vi "06a-arrays.vi"() -> ()   [LabVIEW 2018, in "LV2Julia_examples.lvlib"]
uses:
  LV2Julia_examples.lvlib
  LV2Julia_core/VIs/Server or client state.ctl
  LV2Julia_core/VIs/detailed error info.ctl
  LV2Julia_core/VIs/StackFrame.ctl
  LV2Julia_core/VIs/Commands.ctl
  72a46192-383e-4ee5-9465-71670922b82a.vi
  ef5408d4-6538-41d1-b296-fda05a71e4b0.vi
  5eac2bf2-d9fb-4bf1-948e-1ebc05516bc9.vi
  e4efb182-1b04-4d49-96a3-1defebd055ea.vi
  ebebf057-8b7e-42d1-8726-0ed76f361650.vi
  72a46192-383e-4ee5-9465-71670922b82a.vi/b0d408ed-daf5-454d-9ecc-f8af6744abda.vi
  ef5408d4-6538-41d1-b296-fda05a71e4b0.vi/f9ecc56d-b53d-412a-9af8-1c97b46c8685.vi
  5eac2bf2-d9fb-4bf1-948e-1ebc05516bc9.vi/a7715925-f8ed-4395-a6c4-c44ea2ed31c4.vi
  e4efb182-1b04-4d49-96a3-1defebd055ea.vi/824be71f-c5ad-4223-87c9-7cdbbdd09736.vi
  e4efb182-1b04-4d49-96a3-1defebd055ea.vi/40be3533-35a9-4e4c-8722-5f4375dd3b08.vi
  e4efb182-1b04-4d49-96a3-1defebd055ea.vi/65a45231-dbbd-4efd-9ebd-6183352d96e2.vi
  e4efb182-1b04-4d49-96a3-1defebd055ea.vi/912004ff-3e56-4cd8-9a85-8f939a39ad48.vi
  ebebf057-8b7e-42d1-8726-0ed76f361650.vi/8b08c596-2b3a-4931-825f-803b1b8d8a5d.vi
  ebebf057-8b7e-42d1-8726-0ed76f361650.vi/babf9289-bc17-4402-9d6c-dd341eb03b80.vi
  ebebf057-8b7e-42d1-8726-0ed76f361650.vi/f5e4d7e9-5b25-498c-b19f-44e63bafc011.vi
  ebebf057-8b7e-42d1-8726-0ed76f361650.vi/f575945d-7167-44e6-afc9-6bef2b394933.vi
  72a46192-383e-4ee5-9465-71670922b82a.vi/b0d408ed-daf5-454d-9ecc-f8af6744abda.vi/a9aded84-fb4c-4b99-9bf2-11a6971dcdab.vi
  ef5408d4-6538-41d1-b296-fda05a71e4b0.vi/f9ecc56d-b53d-412a-9af8-1c97b46c8685.vi/e56f9a54-3a9f-4e68-a3a9-7dfa6a6a4783.vi
  5eac2bf2-d9fb-4bf1-948e-1ebc05516bc9.vi/a7715925-f8ed-4395-a6c4-c44ea2ed31c4.vi/ef375900-df6d-41f4-9c7e-1a80cf6f4ef4.vi
  5eac2bf2-d9fb-4bf1-948e-1ebc05516bc9.vi/a7715925-f8ed-4395-a6c4-c44ea2ed31c4.vi/9426179f-6f74-442f-81f5-9a9889e94a31.vi
  5eac2bf2-d9fb-4bf1-948e-1ebc05516bc9.vi/a7715925-f8ed-4395-a6c4-c44ea2ed31c4.vi/92b1a726-e853-4864-8bbd-490dfea2ee44.vi
  e4efb182-1b04-4d49-96a3-1defebd055ea.vi/824be71f-c5ad-4223-87c9-7cdbbdd09736.vi/48639029-375b-4425-8f71-319d45f6e3b4.vi
  e4efb182-1b04-4d49-96a3-1defebd055ea.vi/824be71f-c5ad-4223-87c9-7cdbbdd09736.vi/917fea82-d697-4ce0-a076-0fcf05e30575.vi
  <vilib>/Utility/High Resolution Relative Seconds.vi
  ebebf057-8b7e-42d1-8726-0ed76f361650.vi/8b08c596-2b3a-4931-825f-803b1b8d8a5d.vi/7c704175-0edc-4130-a63e-4578cba14c67.vi
  ebebf057-8b7e-42d1-8726-0ed76f361650.vi/8b08c596-2b3a-4931-825f-803b1b8d8a5d.vi/e3978b93-472d-48a9-bab5-51dddfb91b65.vi
  72a46192-383e-4ee5-9465-71670922b82a.vi/b0d408ed-daf5-454d-9ecc-f8af6744abda.vi/a9aded84-fb4c-4b99-9bf2-11a6971dcdab.vi/7b900d93-8f37-40f8-9be1-02a9d42f9a01.vi
  ef5408d4-6538-41d1-b296-fda05a71e4b0.vi/f9ecc56d-b53d-412a-9af8-1c97b46c8685.vi/e56f9a54-3a9f-4e68-a3a9-7dfa6a6a4783.vi/9a698a4f-3967-4c21-99f3-25ec15178b1d.vi
  e4efb182-1b04-4d49-96a3-1defebd055ea.vi/824be71f-c5ad-4223-87c9-7cdbbdd09736.vi/48639029-375b-4425-8f71-319d45f6e3b4.vi/a5759c25-ed5d-4abc-9007-e1bfd2f512dd.vi
  ebebf057-8b7e-42d1-8726-0ed76f361650.vi/8b08c596-2b3a-4931-825f-803b1b8d8a5d.vi/7c704175-0edc-4130-a63e-4578cba14c67.vi/0dcbc56f-df0e-4a08-a62c-191f3a396a75.vi
  LV2Julia_core/VIs/jl-scripts path.vi
  LV2Julia_core/VIs/check ID validity.vi
  LV2Julia_core/VIs/bindata_descr to JSON.vi
  LV2Julia_core/VIs/check cluster field names.vi
  LV2Julia_core/VIs/concat JSON.vi
  LV2Julia_core/VIs/build request.vi
  LV2Julia_core/VIs/Parse server response.vi
  LV2Julia_core/VIs/log jl exceptions.vi
  <vilib>/Utility/error.llb/Error Cluster From Error Code.vi
  LV2Julia_core/LV2Julia_core.lvlib
panel:
  in  "invert matrix":cluster{"invert":bool}={"invert"=TRUE}
  out "inverted matrix":dbl[][](array[numeric])=[[1.0, 0.0, 5.0], [4.0, 2.0, 1.0], [2.0, 2.0, 3.0]] format="%#.4g"
  out "determinant":dbl
  out "Solution Vector":dbl[](array[numeric]) format="%.2f"
  in  "Known Vector":dbl[](array[numeric])=[22.0, 14.0, 18.0]
  in  "Input Matrix":dbl[][](array[numeric])=[[1.0, 0.0, 5.0], [4.0, 2.0, 1.0], [2.0, 2.0, 3.0]]
  in  "next":bool
  out "detailed error info":T1
  out "current error":errorcluster
  out "final error":errorcluster
  out "short err code":u8
  in  "stop":bool
  out "ZMQ timeout":bool
  out "Julia script file path":path
  out "temporary script path":path
  out "Jl Server state":T3
  # "A Bool scalar, a 2D and a 1D array of Float are sent as arguments. \n\nA 1D array and optionally a 2D array and a scalar are returned."
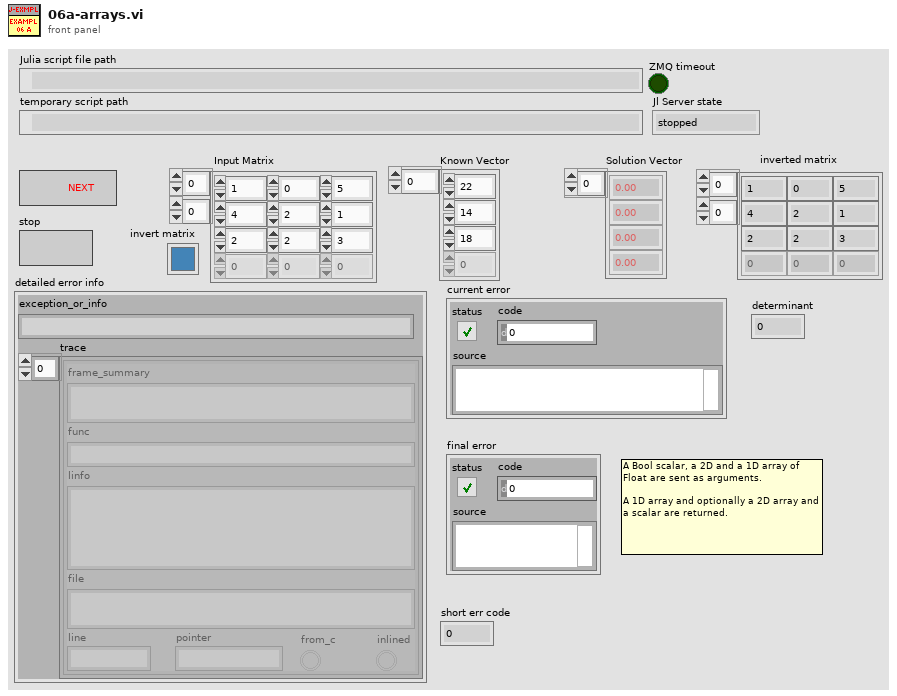
[diagram p1: front panel]
types:
  T1 = typedef "LV2Julia_core.lvlib/detailed error info.ctl" = cluster{"exception_or_info":string, "trace":T2[]}
  T2 = typedef "LV2Julia_core.lvlib/StackFrame.ctl" = cluster{"frame_summary":string, "func":string, "linfo":string, "file":string, "line":i32, "pointer":u64, "from_c":bool, "inlined":bool}
  T3 = typedef "LV2Julia_core.lvlib/Server or client state.ctl" = enum16{"stopped", "running", "unknown"}
  T4 = typedef "LV2Julia_core.lvlib/Commands.ctl" = enum16{"Start Jl-server & Init LV-client", "Send request & Get response ", "Stop Jl-server & Cleanup LV-client", "Cleanup LV-client", "Start Jl-server", "Stop Jl-server", "Init LV-Client", "Cleanup LV-Client", "(not allowed)", "Set LV Client state", "Set Jl Server state", "set ZMQ timeout", "read ZMQ timeout", "read-out state"}
  T5 = typedef "LV2Julia_core.lvlib/Bindata&description.ctl" = cluster{"bindata_descr":T6[], "bindata":u8[]}
  T6 = typedef "LV2Julia_core.lvlib/Bindata description.ctl" = cluster{"nofbytes":i32, "numtype":string, "start":i32, "arrdims":i32[], "kwarg_name":string, "category":string}
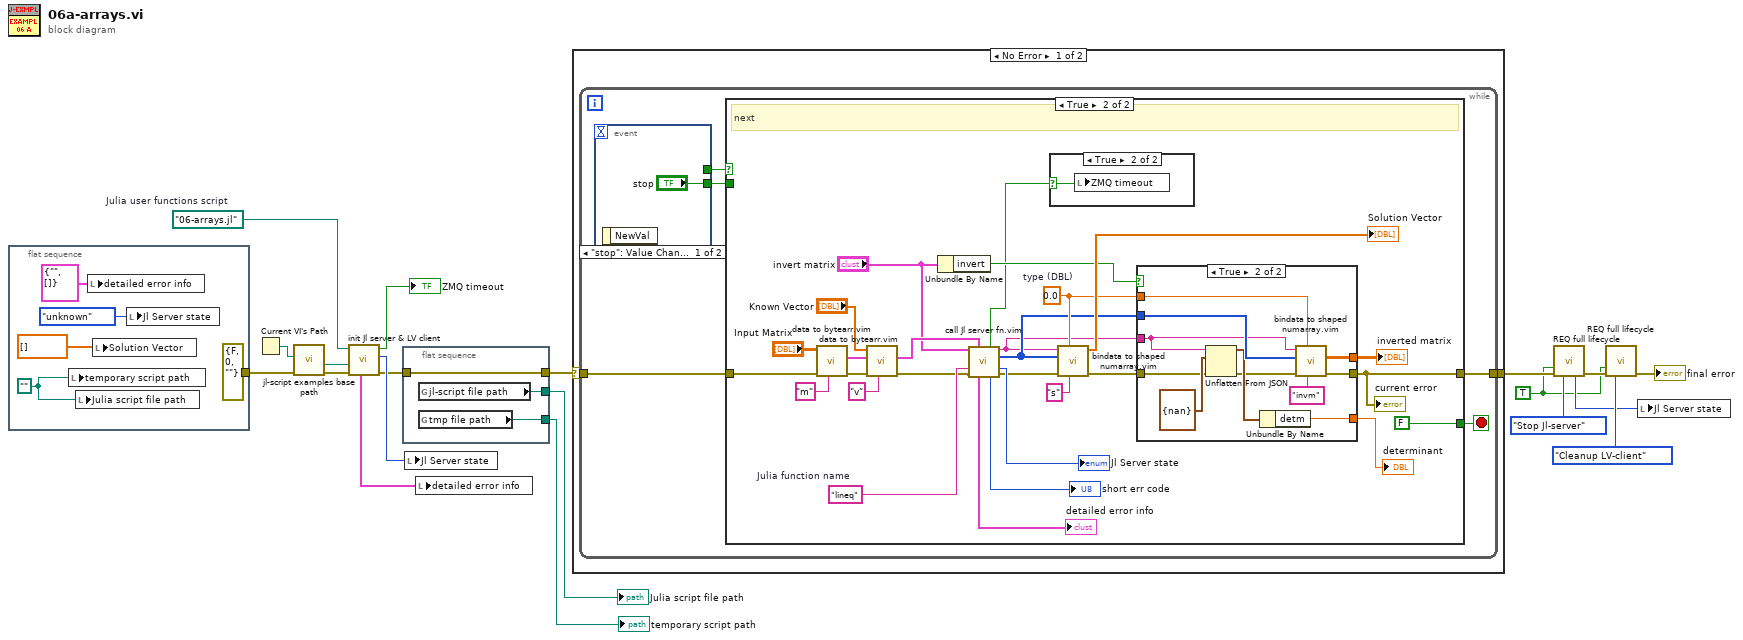
[diagram p0: block diagram]
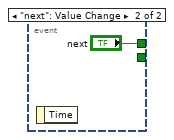
[diagram p2: hidden frame]
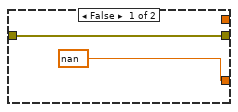
[diagram p4: hidden frame]
diagram:
  w9 = path "06-arrays.jl"  # Julia user functions script
  w10 = TRUE ("Force command")
  n1 = flat-sequence {
    tunnel: [errorcluster {"status"=FALSE, "code"=0, "source"=""} ("error in (no error)")] -> w2
    frame #0 {
      w20 = path ""
      n2 = local write "temporary script path"(w20) -> ()
      n3 = local write "Julia script file path"(w20) -> ()
      n4 = local write "detailed error info"(T1 {"exception_or_info"="", "trace"=[]} ("detailed error info")) -> ()
      n5 = local write "Solution Vector"(dbl[] [] ("Server response")) -> ()
      n6 = local write "Jl Server state"(Server_or_client_state."unknown" ("Jl Server state out")) -> ()
    }
  }
  n7 = Current VI's Path() -> (path=w5:path)
  n8 = call "jl-script examples base path.vi"("error in (no error)"=w2, "calling example VI path"=w5) -> ("error out"=w4:errorcluster, "jl-script-examples base path"=w3:path)  [unwired: 8 in]
  n9 = call "init Jl server & LV client.vi"("error in (no error)"=w4, "Base path (not a path)"=w3, "Julia user functions script"=w9) -> ("error out"=w6:errorcluster, "Jl Server state out"=w7:T3, "timeout?"=→"ZMQ timeout":bool, "detailed error info"=w1:T1)  [unwired: 3 in, 2 out]
  n10 = flat-sequence {
    tunnel: [w27] -> w14
    tunnel: w6 -> [w27]
    tunnel: [w26] -> w12
    tunnel: [w25] -> w13
    frame #0 {
      n11 = global read "jl-scripts path.vi" "jl-script file path"() -> (w26:path)
      n12 = global read "jl-scripts path.vi" "tmp file path"() -> (w25:path)
    }
  }
  n13 = local write "Jl Server state"(w7) -> ()
  n14 = local write "detailed error info"(w1) -> ()
  n15 = case shown="No Error" w14 {
    selector: w14 -> [w28 w80]
    tunnel: [w29 w80] -> w19
    frame No Error {
      n16 = while {
        tunnel: w28 -> [w33]
        tunnel: [w34] -> w29
        stop <- w31 stop-if-true
        n17 = event shown="[0] \"stop\": Value Change" {
          selector: _ -> [_ _]
          dyn-events: _ -> [_ _]
          timeout: _ -> [_ _]
          tunnel: [_ "next"] -> w32
          tunnel: ["stop" _] -> w30
          event "stop": Value Change {
            n18 = event-data() -> ()  [unwired: 1 in, 1 out]
          }
          event "next": Value Change {
            n19 = event-data() -> ()  [unwired: 1 in, 1 out]
          }
        }
        n20 = case shown="True" w32 {
          tunnel: [w38 w45] -> w34
          tunnel: w33 -> [w38 w60]
          tunnel: [w37 FALSE ("stop this VI only")] -> w31
          tunnel: w30 -> [w37 _]
          frame False {
            # "stop"
          }
          frame True {
            w55 = 0.0  # type (DBL)
            w49 = "lineq"  # Julia function name
            # "next"
            n21 = call "data to bytearr.vim"("kwarg_name"="m", "error in (no error)"=w60, "data in"="Input Matrix") -> ("error out"=w63:errorcluster, "Bindata & descr out"=w62:T5)  [unwired: 6 in, 1 out]
            n22 = call "data to bytearr.vim"("kwarg_name"="v", "error in (no error)"=w63, "Bindata & descr in"=w62, "data in"="Known Vector") -> ("error out"=w48:errorcluster, "Bindata & descr out"=w47:T5)  [unwired: 5 in, 1 out]
            n23 = Unbundle By Name("invert matrix") -> ("invert"=w43:bool)
            n24 = call "call Jl server fn.vim"("Arguments 1"="invert matrix", "Bindata & descr in"=w47, "fun2call"=w49, "error in (no error)"=w48) -> ("timeout?"=w42:bool, "JSON received"=w41:string, "binary data received"=w46:u8[], "Jl Server state out"=→"Jl Server state":T3, "detailed error info"=→"detailed error info":T1, "return code"=→"short err code":u8, "error out"=w50:errorcluster)  [unwired: 5 in]
            n25 = case shown="True" w42 {
              selector: w42 -> [_ w79]
              frame False {
              }
              frame True {
                n26 = local write "ZMQ timeout"(w79) -> ()
              }
            }
            n27 = call "bindata to shaped numarray.vim"("name"="s" ("kwarg_name"), "element type"=w55, "error in (no error)"=w50, "binary data"=w46, "JSON in"=w41) -> ("error out"=w40:errorcluster, "numarray 1D"=→"Solution Vector":dbl[])  [unwired: 1 in, 4 out]
            n28 = case shown="True" w43 {
              tunnel: w55 -> [_ w77]
              tunnel: [_ w76] -> w54
              tunnel: w46 -> [_ w75]
              tunnel: w41 -> [_ w69]
              tunnel: [w67 w74] -> w45
              tunnel: w40 -> [w67 w72]
              tunnel: [nan ("detm") w68] -> w39
              frame False {
              }
              frame True {
                n29 = Unflatten From JSON(JSON string=w69, type and defaults=cluster{"detm":dbl} {"detm"=nan}, error in (no error)=w72) -> (value=w71:cluster{"detm":dbl}, error out=w70:errorcluster)  [unwired: 4 in]
                n30 = Unbundle By Name(w71) -> ("detm"=w68:dbl)
                n31 = call "bindata to shaped numarray.vim"("name"="invm" ("kwarg_name"), "element type"=w77, "error in (no error)"=w70, "binary data"=w75, "JSON in"=w69) -> ("error out"=w74:errorcluster, "numarray 2D"=w76:dbl[][])  [unwired: 1 in, 4 out]
              }
            }
            "current error" <- w45
            "inverted matrix" <- w54
            "determinant" <- w39
          }
        }
      }
    }
    frame Error {
    }
  }
  n32 = call "REQ full lifecycle.vi"("Force command"=w10, "error in"=w19, "command"=Commands."Stop Jl-server") -> ("Jl Server state out"=w11:T3, "error out"=w17:errorcluster)  [unwired: 6 in, 5 out]
  n33 = call "REQ full lifecycle.vi"("Force command"=w10, "error in"=w17, "command"=Commands."Cleanup LV-client") -> ("error out"=→"final error":errorcluster)  [unwired: 6 in, 6 out]
  n34 = local write "Jl Server state"(w11) -> ()
  "temporary script path" <- w13
  "Julia script file path" <- w12
